vi "Register Input Request.vi"(8 "error in":errorcluster, 9 "requestedSchema":string, 10 "message":string, 11 "key":string) -> (0 "error out":errorcluster)   [LabVIEW 2020, in "MCP Server.lvlib"]
doc: "Registers one question of Ask User.vi for the result of the running tools/call: enqueues {\"<key>\":{\"method\":\"elicitation/create\",\"params\":{\"mode\":\"form\",\"message\":..,\"requestedSchema\":..}}} on the named queue \"MCP Input Requests\", which Collect MCP Input Requests.vi turns into the inputRequests of an input_required result.\n\nrequestedSchema is passed on as given when it is a JSON object; empty or anything else is replaced by {\"type\":\"object\",\"properties\":{}} (a plain confirmation).\n\nRuns regardless of error in; error out is error in merged with the errors of the queue operations."
uses:
  MCP Server.lvlib
  ae42319d-1f10-4334-9c73-cae60571a2b3.vi
  1e81a64f-11f2-4b84-97bb-0fd0b20cdda2.vi
  <vilib>/JDP Science/JSONtext/Variant to JSON Text.vi
  <vilib>/JDP Science/JSONtext/LVClass Serializer/JSONtext LVClass Serializer.lvclass
  <vilib>/JDP Science/JSONtext/JSONtext.lvlib
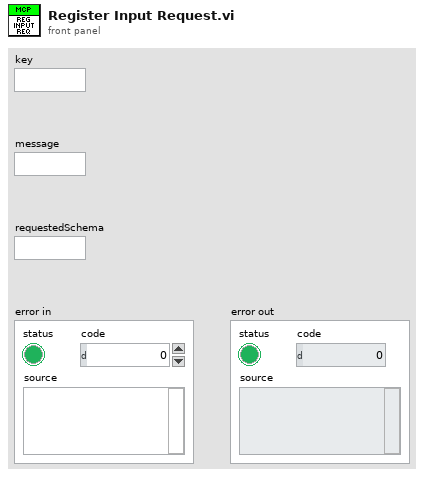
[diagram p1: front panel]
types:
  T1 = typedef "JSONtext.lvlib/JSON Value Type.ctl" = enum16{"Not a JSON Value", "JSON Object", "JSON Array", "String", "Number", "true", "false", "null"}
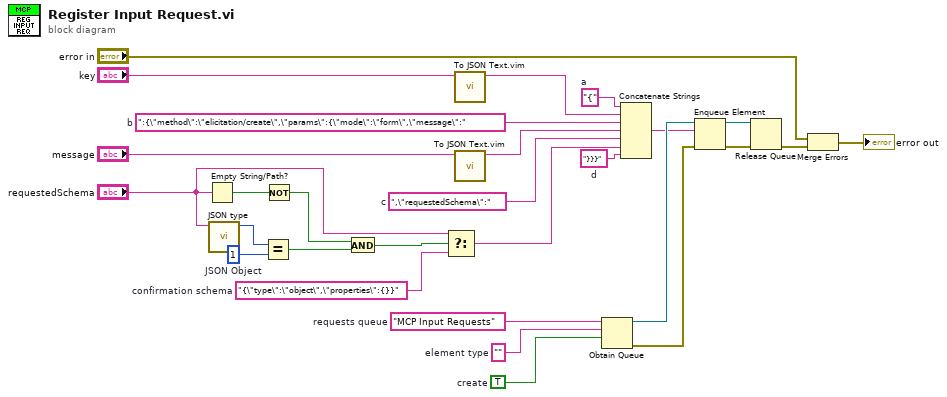
[diagram p0: block diagram]
diagram:
  w12 = "}}}"  # d
  w14 = ",\"requestedSchema\":"  # c
  w16 = ":{\"method\":\"elicitation/create\",\"params\":{\"mode\":\"form\",\"message\":"  # b
  w18 = "{"  # a
  w19 = "{\"type\":\"object\",\"properties\":{}}"  # confirmation schema
  w24 = u16 1  # JSON Object
  w9 = TRUE  # create
  w10 = ""  # element type
  w11 = "MCP Input Requests"  # requests queue
  n1 = Empty String/Path?(string/path="requestedSchema") -> (empty?=w26:bool)
  n2 = call <vilib>:"JSON type.vi"("JSON"="requestedSchema") -> ("JSON Value Type"=w25:T1)  [unwired: 9 in, 1 out]
  n3 = Equal?(x=w25, y=w24) -> (x = y?=w22:bool)
  n4 = Not(x=w26) -> (.not. x?=w23:bool)
  n5 = And(x=w23, y=w22) -> (x .and. y?=w20:bool)
  n6 = Select(t="requestedSchema", s=w20, f=w19) -> (s? t:f=w13:string)
  n7 = call "To JSON Text.vim"("Anything"="key") -> ("<JSON>"=w17:string)  [unwired: 9 in, 1 out]
  n8 = call "To JSON Text.vim"("Anything"="message") -> ("<JSON>"=w15:string)  [unwired: 9 in, 1 out]
  n9 = Obtain Queue(name (unnamed)=w11, element data type=w10, create if not found? (T)=w9) -> (queue out=w8:refnum<queue>, error out=w6:errorcluster)  [unwired: 2 in, 1 out]
  n10 = Concatenate Strings(w18, w17, w16, w15, w14, w13, w12) -> (w7:string)
  n11 = Enqueue Element(queue=w8, element=w7, error in (no error)=w6) -> (queue out=w5:refnum<queue>, error out=w4:errorcluster)  [unwired: 1 in, 1 out]
  n12 = Release Queue(queue=w5, error in (no error)=w4) -> (error out=w2:errorcluster)  [unwired: 1 in, 2 out]
  n13 = Merge Errors("error in", w2) -> (→"error out":errorcluster)
